vi "setup_process_queues.vi"(11 "Tool Assignments":T1) -> (0 "Process queue names out":string[](array[string]), 3 "Process queues":refnum<queue>[](array[refnum]))   [LabVIEW 2017, in "labview-standard-library.lvlib" / "automode-scripting.lvlib"]
uses:
  automode-scripting.lvlib
  type-defs/command_line_info.ctl
  type-defs/tool-assignments.ctl
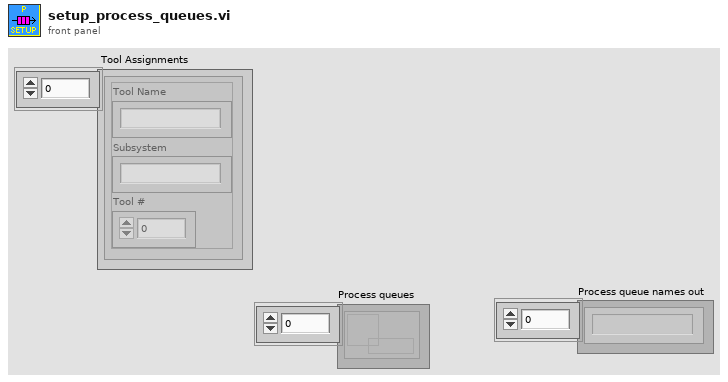
[diagram p1: front panel]
types:
  T1 = typedef "tool-assignments.ctl" = cluster{"Tool Name":string, "Subsystem":string, "Tool #":i32}[]
  T2 = typedef "labview-standard-library.lvlib/automode-scripting.lvlib/command_line_info.ctl" = cluster{"Line text":string, "Line #":i32}
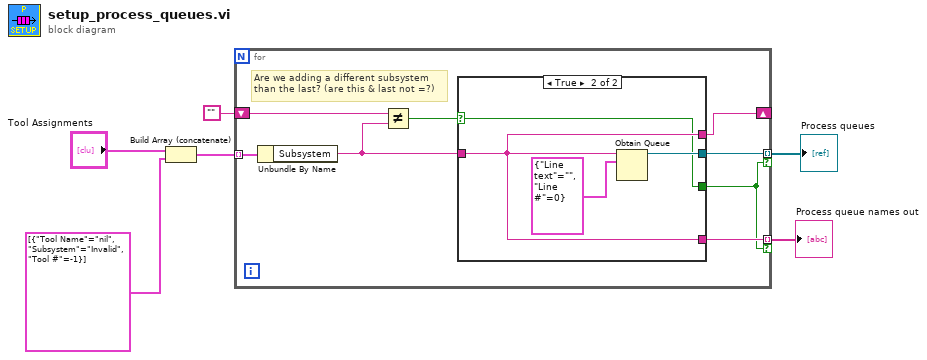
[diagram p0: block diagram]
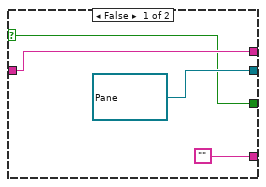
[diagram p2: hidden frame]
diagram:
  n1 = Build Array (concatenate)("Tool Assignments", T1 [{"Tool Name"="nil", "Subsystem"="Invalid", "Tool #"=-1}] ("Tool Assignments 2")) -> (w2:T1)
  n2 = for {
    tunnel: w2 -> [w13] mode=indexing
    tunnel: [w14] -> w6 mode=indexing if=w7
    tunnel: [w11] -> w4 mode=indexing if=w7
    shift-right: [w8] -> _
    shift-left: "" -> [w12]
    # "Are we adding a different subsystem\nthan the last? (are this & last not =?)"
    n3 = Unbundle By Name(w13) -> ("Subsystem"=w9:string)
    n4 = Not Equal?(x=w12, y=w9) -> (x != y?=w10:bool)
    n5 = case shown="True" w10 {
      selector: w10 -> [w15 w19]
      tunnel: [refnum<queue> refnum ("queue out") w22] -> w14
      tunnel: w9 -> [w17 w20]
      tunnel: ["" w20] -> w11
      tunnel: [w17 w20] -> w8
      tunnel: [w15 w19] -> w7
      frame False {
      }
      frame True {
        n6 = Obtain Queue(name (unnamed)=w20, element data type=T2 {"Line text"="", "Line #"=0}) -> (queue out=w22:refnum<queue>)  [unwired: 3 in, 2 out]
      }
    }
  }
  "Process queues" <- w6
  "Process queue names out" <- w4
